vi "update Keysight 9020A Correction Table Param.vi"(8 "error in (no error)":errorcluster, 10 "Keysight Correction Table":T1 {"Frequency (Hz)" format="%#_6p"}, 11 "Keysight 9020A in":refnum<class "Keysight 9020A.lvclass">) -> (0 "error out":errorcluster, 3 "Keysight 9020A out":refnum<class "Keysight 9020A.lvclass">)   [LabVIEW 2023, in "Spectrum Analyzer.lvlib" / "Keysight 9020A.lvclass"]
uses:
  Keysight 9020A.lvclass
  TYPE DEFINITION/Keysight 9020A/TYPE Keysight Correction Table Array.ctl
  Keysight 9020A.lvclass/Keysight 9020A.ctl
  Spectrum Analyzer.lvlib
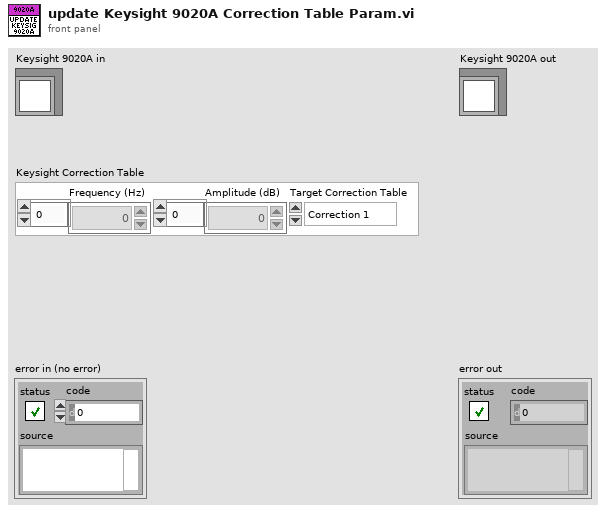
[diagram p1: front panel]
types:
  T1 = typedef "Spectrum Analyzer.lvlib/TYPE Keysight Correction Table Array.ctl" = cluster{"Frequency (Hz)":dbl[], "Amplitude (dB)":dbl[], "Target Correction Table":enum16{"Correction 1", "Correction 2", "Correction 3", "Correction 4", "Correction 5", "Correction 6", "Correction 7", "Correction 8"}}
  T2 = enum16{"Correction 1", "Correction 2", "Correction 3", "Correction 4", "Correction 5", "Correction 6", "Correction 7", "Correction 8"}
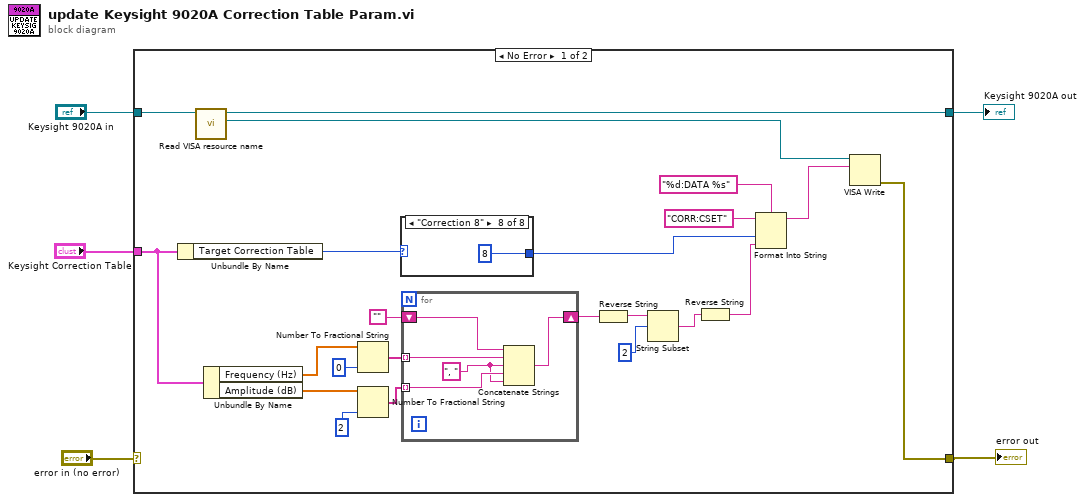
[diagram p0: block diagram]
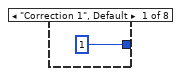
[diagram p2: hidden frame]
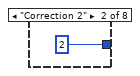
[diagram p3: hidden frame]
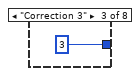
[diagram p4: hidden frame]
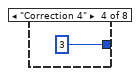
[diagram p5: hidden frame]
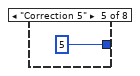
[diagram p6: hidden frame]
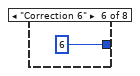
[diagram p7: hidden frame]
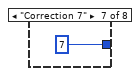
[diagram p8: hidden frame]
diagram:
  n1 = case shown="No Error" "error in (no error)" {
    selector: "error in (no error)" -> [_ w42]
    tunnel: [w27 w41] -> w5
    tunnel: [w23 w42] -> w2
    tunnel: "Keysight 9020A in" -> [w21 w41]
    tunnel: "Keysight Correction Table" -> [w18 _]
    frame No Error {
      n2 = Unbundle By Name(w18) -> ("Target Correction Table"=w20:T2)
      n3 = call "Read VISA resource name.vi"("Keysight 9020A in"=w21) -> ("VISA resource name"=w22:refnum<visa-resource-name>, "Keysight 9020A out"=w27:refnum<class "Keysight 9020A.lvclass">)  [unwired: 8 in, 1 out]
      n4 = Unbundle By Name(w18) -> ("Frequency (Hz)"=w17:dbl[], "Amplitude (dB)"=w14:dbl[])
      n5 = Number To Fractional String(number=w17, precision (6)=i16 0) -> (F-format string=w16:string[])  [unwired: 2 in]
      n6 = Number To Fractional String(number=w14, precision (6)=i16 2) -> (F-format string=w12:string[])  [unwired: 2 in]
      n7 = case shown="\"Correction 8\"" w20 {
        tunnel: [1 2 3 3 5 6 7 8] -> w19
        frame "Correction 1", Default {
        }
        frame "Correction 2" {
        }
        frame "Correction 3" {
        }
        frame "Correction 4" {
        }
        frame "Correction 5" {
        }
        frame "Correction 6" {
        }
        frame "Correction 7" {
        }
        frame "Correction 8" {
        }
      }
      n8 = for {
        tunnel: w16 -> [w32] mode=indexing
        tunnel: w12 -> [w30] mode=indexing
        shift-right: [w28] -> w10
        shift-left: "" -> [w31]
        w29 = ", " ("string")
        n9 = Concatenate Strings(w31, w32, w29, w30, w29) -> (w28:string)
      }
      n10 = Reverse String(1:w10) -> (0:w9:string)
      n11 = String Subset(string=w9, offset (0)=2) -> (substring=w7:string)  [unwired: 1 in]
      n12 = Reverse String(1:w7) -> (0:w6:string)
      n13 = Format Into String(format string="%d:DATA %s", initial string="CORR:CSET", w19, w6) -> (resulting string=w24:string)  [unwired: 1 in, 1 out]
      n14 = VISA Write(VISA resource name=w22, write buffer=w24) -> (error out=w23:errorcluster)  [unwired: 1 in, 2 out]
    }
    frame Error {
    }
  }
  "error out" <- w2
  "Keysight 9020A out" <- w5
